vi "VIH HelpGen - HTML - Build A HREF Tag to Email.vi"(7 "Escape Reserved HTML chars in body (F)":bool, 10 "Subject":string, 11 "Email address":string) -> (3 "HTML tag":string)   [LabVIEW 2014]
doc: "::: VI Helpeks :::\nCopyright (c) 2000-2026 Konstantin Shifershteyn. All rights reserved."
panel:
  # "VI Helpeks\nCopyright (c) 2012-2026 Konstantin Shifershteyn"
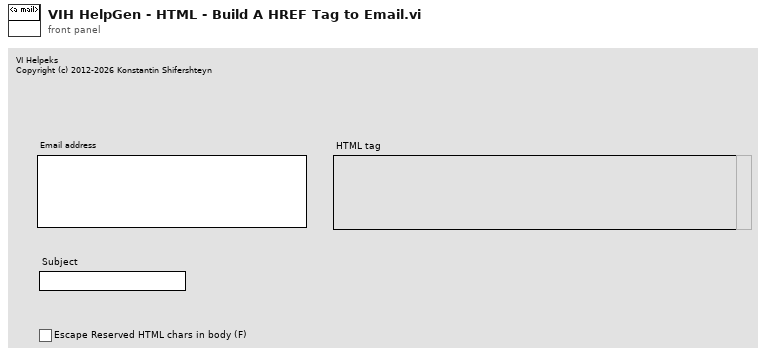
[diagram p1: front panel]
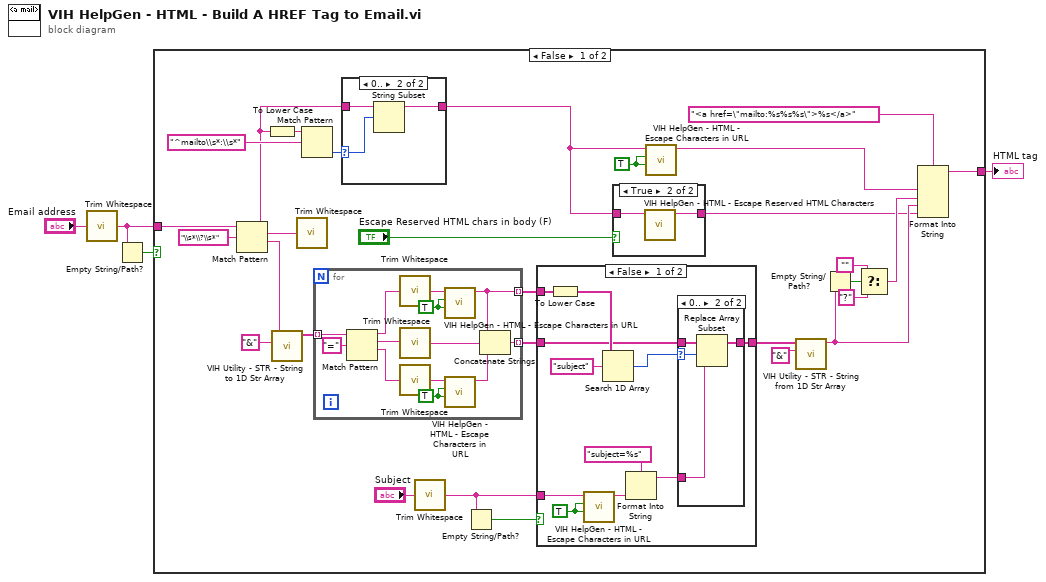
[diagram p0: block diagram]
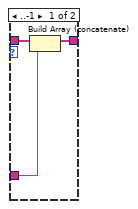
[diagram p4: hidden frame]
diagram:
  n1 = call <vilib>:"Trim Whitespace.vi"("string"="Email address") -> ("trimmed string"=w1:string)  [unwired: 1 in]
  n2 = Empty String/Path?(string/path=w1) -> (empty?=w2:bool)
  n3 = case shown="False" w2 {
    tunnel: [w28 w73] -> w4
    tunnel: w1 -> [w26 w73]
    frame False {
      w27 = TRUE
      n4 = Match Pattern(string=w26, regular expression="\\s*\\?\\s*") -> (before substring=w7:string, match substring=w31:string, after substring=w25:string)  [unwired: 1 in, 1 out]
      n5 = To Lower Case(string=w7) -> (all lower case string=w9:string)
      n6 = call "VIH Utility - STR - String to 1D Str Array.vi"("delimiter ('\\n')"="&" ("delimiter ('\\n')"), "String in"=w25) -> ("Array out"=w23:string[])  [unwired: 5 in]
      n7 = call <vilib>:"Trim Whitespace.vi"("string"=w31) -> ()  [unwired: 1 in, 1 out]
      n8 = Match Pattern(string=w9, regular expression="^mailto\\s*:\\s*") -> (offset past match=w8:i32)  [unwired: 1 in, 3 out]
      n9 = for {
        tunnel: w23 -> [w52] mode=indexing
        tunnel: [w44] -> w22 mode=indexing
        tunnel: [w41] -> w13 mode=indexing
        w48 = TRUE
        w49 = TRUE
        n10 = Match Pattern(string=w52, regular expression="=") -> (before substring=w47:string, match substring=w51:string, after substring=w46:string)  [unwired: 1 in, 1 out]
        n11 = call <vilib>:"Trim Whitespace.vi"("string"=w47) -> ("trimmed string"=w43:string)  [unwired: 1 in]
        n12 = call <vilib>:"Trim Whitespace.vi"("string"=w51) -> ("trimmed string"=w50:string)  [unwired: 1 in]
        n13 = call <vilib>:"Trim Whitespace.vi"("string"=w46) -> ("trimmed string"=w42:string)  [unwired: 1 in]
        n14 = call "VIH HelpGen - HTML - Escape Characters in URL.vi"("Escape mailto Reserved chars (F)"=w49, "Escape HTML Reserved chars (T)"=w49, "string"=w43) -> ("URL string"=w41:string)  [unwired: 8 in]
        n15 = call "VIH HelpGen - HTML - Escape Characters in URL.vi"("Escape mailto Reserved chars (F)"=w48, "Escape HTML Reserved chars (T)"=w48, "string"=w42) -> ("URL string"=w45:string)  [unwired: 8 in]
        n16 = Concatenate Strings(w41, w50, w45) -> (w44:string)
      }
      n17 = case shown="0.." w8 {
        selector: w8 -> [_ w36]
        tunnel: w7 -> [w34 w37]
        tunnel: [w34 w35] -> w6
        frame ..-1 {
        }
        frame 0.. {
          n18 = String Subset(string=w37, offset (0)=w36) -> (substring=w35:string)  [unwired: 1 in]
        }
      }
      n19 = call <vilib>:"Trim Whitespace.vi"("string"="Subject") -> ("trimmed string"=w5:string)  [unwired: 1 in]
      n20 = Empty String/Path?(string/path=w5) -> (empty?=w29:bool)
      n21 = case shown="False" w29 {
        tunnel: w5 -> [w63 _]
        tunnel: w22 -> [w54 w72]
        tunnel: [w59 w72] -> w21
        tunnel: w13 -> [w58 _]
        frame False {
          w61 = TRUE
          n22 = To Lower Case(string=w58) -> (all lower case string=w57:string[])
          n23 = call "VIH HelpGen - HTML - Escape Characters in URL.vi"("Escape mailto Reserved chars (F)"=w61, "Escape HTML Reserved chars (T)"=w61, "string"=w63) -> ("URL string"=w62:string)  [unwired: 8 in]
          n24 = Search 1D Array(1D array=w57, element="subject" ("format string")) -> (index of element=w55:i32)  [unwired: 1 in]
          n25 = Format Into String(format string="subject=%s", w62) -> (resulting string=w60:string)  [unwired: 2 in, 1 out]
          n26 = case shown="0.." w55 {
            selector: w55 -> [_ w68]
            tunnel: w60 -> [w67 w69]
            tunnel: [w66 w70] -> w59
            tunnel: w54 -> [w65 w71]
            frame ..-1 {
              n27 = Build Array (concatenate)(w65, w67) -> (w66:string[])
            }
            frame 0.. {
              n28 = Replace Array Subset(array=w71, new element=w69, index=w68) -> (w70:string[])
            }
          }
        }
        frame True {
        }
      }
      n29 = case shown="True" "Escape Reserved HTML chars in body (F)" {
        tunnel: w6 -> [w38 w40]
        tunnel: [w38 w39] -> w12
        frame False {
        }
        frame True {
          n30 = call "VIH HelpGen - HTML - Escape Reserved HTML Characters.vi"("string"=w40) -> ("HTML string"=w39:string)  [unwired: 10 in]
        }
      }
      n31 = call "VIH HelpGen - HTML - Escape Characters in URL.vi"("Escape mailto Reserved chars (F)"=w27, "Escape HTML Reserved chars (T)"=w27, "string"=w6) -> ("URL string"=w19:string)  [unwired: 8 in]
      n32 = call "VIH Utility - STR - String from 1D Str Array.vi"("delimiter ('\\n')"="&" ("delimiter ('\\n')"), "Array in"=w21) -> ("String out"=w15:string)  [unwired: 5 in]
      n33 = Empty String/Path?(string/path=w15) -> (empty?=w18:bool)
      n34 = Select(t="", s=w18, f="?") -> (s? t:f=w14:string)
      n35 = Format Into String(format string="<a href=\"mailto:%s%s%s\">%s</a>", w19, w14, w15, w12) -> (resulting string=w28:string)  [unwired: 2 in, 1 out]
    }
    frame True {
    }
  }
  "HTML tag" <- w4
